vi "init Jl server & LV client.vi"(8 "error in (no error)":errorcluster, 9 "Base path (not a path)":path=path "", 11 "Julia user functions script":path) -> (0 "error out":errorcluster, 2 "Jl Server state out":T4, 3 "timeout?":bool, 4 "return code":u8, 5 "LVServer_version":T1, 6 "detailed error info":T2)   [LabVIEW 2018, in "LV2Julia_core.lvlib"]
doc: "Init Julia server & LabView client."
uses:
  LV2Julia_core.lvlib
  Server or client state.ctl
  detailed error info.ctl
  StackFrame.ctl
  VersionNumber.ctl
  Commands.ctl
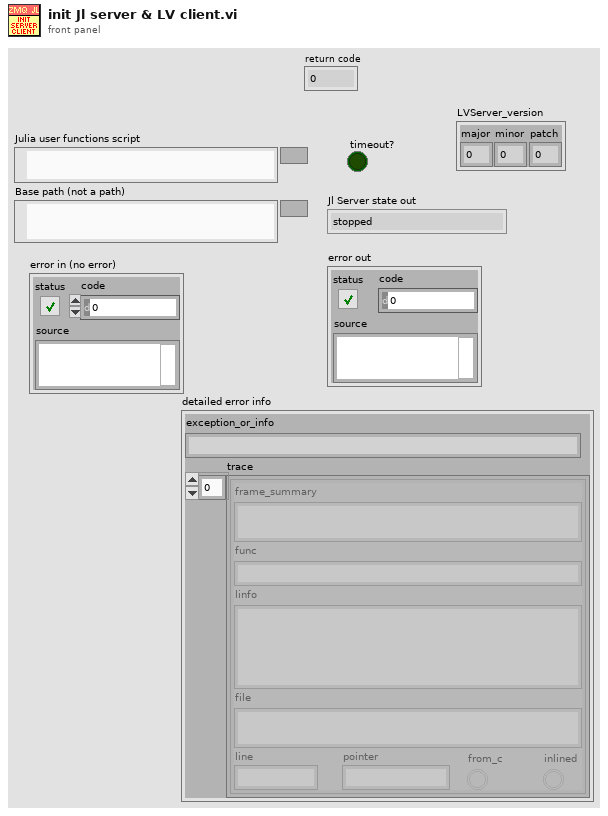
[diagram p1: front panel]
types:
  T1 = typedef "LV2Julia_core.lvlib/VersionNumber.ctl" = cluster{"major":u16, "minor":u16, "patch":u16}
  T2 = typedef "LV2Julia_core.lvlib/detailed error info.ctl" = cluster{"exception_or_info":string, "trace":T3[]}
  T3 = typedef "LV2Julia_core.lvlib/StackFrame.ctl" = cluster{"frame_summary":string, "func":string, "linfo":string, "file":string, "line":i32, "pointer":u64, "from_c":bool, "inlined":bool}
  T4 = typedef "LV2Julia_core.lvlib/Server or client state.ctl" = enum16{"stopped", "running", "unknown"}
  T5 = typedef "LV2Julia_core.lvlib/Commands.ctl" = enum16{"Start Jl-server & Init LV-client", "Send request & Get response ", "Stop Jl-server & Cleanup LV-client", "Cleanup LV-client", "Start Jl-server", "Stop Jl-server", "Init LV-Client", "Cleanup LV-Client", "(not allowed)", "Set LV Client state", "Set Jl Server state", "set ZMQ timeout", "read ZMQ timeout", "read-out state"}
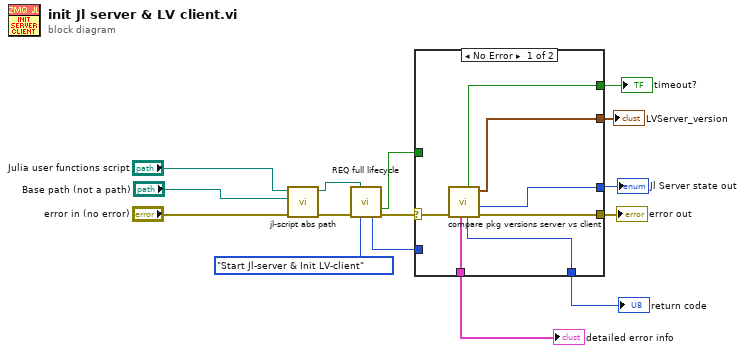
[diagram p0: block diagram]
diagram:
  n1 = call "jl-script abs path.vi"("error in (no error)"="error in (no error)", "Base path (not a path)"="Base path (not a path)", "Julia user functions script"="Julia user functions script") -> ("error out"=w7:errorcluster, "script abs path"=w6:path)  [unwired: 7 in]
  n2 = call "REQ full lifecycle.vi"("Julia user functions script"=w6, "error in"=w7, "command"=Commands."Start Jl-server & Init LV-client") -> ("timeout?"=w11:bool, "Jl Server state out"=w14:T4, "error out"=w10:errorcluster)  [unwired: 6 in, 4 out]
  n3 = case shown="No Error" w10 {
    selector: w10 -> [w22 w24]
    tunnel: [w20 w25] -> w12
    tunnel: w11 -> [_ w25]
    tunnel: [w21 w24] -> w13
    tunnel: [w19 w23] -> w15
    tunnel: w14 -> [_ w23]
    tunnel: [w18 _] -> w3
    tunnel: [w17 _] -> w2
    tunnel: [w16 _] -> w1
    frame No Error {
      n4 = call "compare pkg versions server vs client.vi"("error in (no error)"=w22) -> ("error out"=w21:errorcluster, "Jl Server state out"=w19:T4, "LVServer_version"=w16:T1, "return code"=w17:u8, "timeout?"=w20:bool, "detailed error info"=w18:T2)  [unwired: 5 in]
    }
    frame Error {
    }
  }
  "Jl Server state out" <- w15
  "error out" <- w13
  "timeout?" <- w12
  "detailed error info" <- w3
  "return code" <- w2
  "LVServer_version" <- w1
